vi "Load test file.vi"() -> (1 "Voltaje del detector [V]":dbl[](array[numeric]), 2 "Corriente [mA]":dbl[](array[numeric]), 3 "Voltaje [V]":dbl[](array[numeric]))   [LabVIEW 2020]
uses:
  controls/Graph data --typedef.ctl
  <vilib>/Utility/file.llb/Read Delimited Spreadsheet (DBL).vi
panel:
  out "Eficiencia luminosa-V":cluster{dbl[], dbl[]}(graph) caption="L-V"
  out "Eficiencia de corriente-V":cluster{dbl[], dbl[]}(graph) caption="L-V"
  out "J-V":cluster{dbl[], dbl[]}(graph)
  out "L-V":cluster{dbl[], dbl[]}(graph)
  out "Graph data":T1
  out "Eficiencia luminosa [lm/W]":dbl[](array[numeric])
  out "Eficiencia de corriente [Cd/A]":dbl[](array[numeric])
  out "Luminancia [Cd/m2]":dbl[](array[numeric])
  out "Iluminancia [Lux]":dbl[](array[numeric])
  out "Densidad de corriente [mA/cm2]":dbl[](array[numeric])
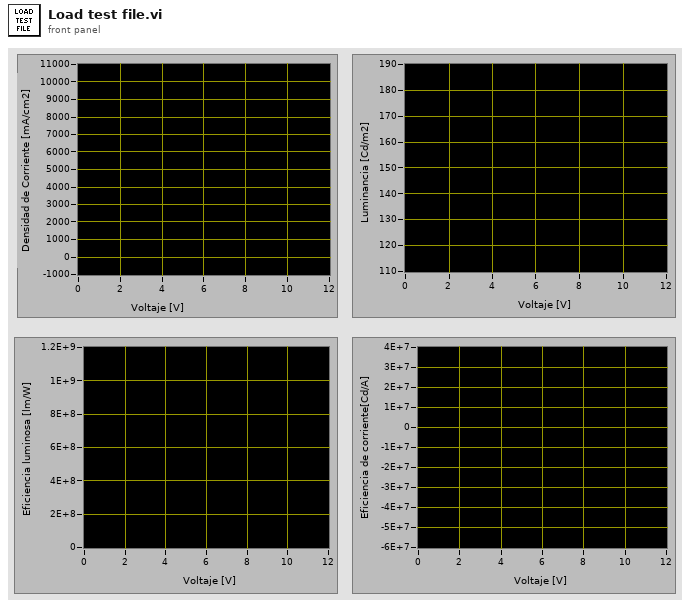
[diagram p1: front panel]
types:
  T1 = typedef "Graph data --typedef.ctl" = cluster{"Voltaje [V]":dbl[], "Corriente [mA]":dbl[], "Densidad de corriente [CD/A]":dbl[], "Iluminancia [Lm/m2]":dbl[], "Luminance [Cd/m2]":dbl[], "Ef corriente [Cd/A]":dbl[], "Ef Luminosa [Cd/W]":dbl[], "V detector [V]":dbl[], "Pin [W]":dbl[]}
  T2 = cluster{"Voltaje [V]":dbl[], "Densidad de corriente [CD/A]":dbl[]}
  T3 = cluster{"Voltaje [V]":dbl[], "Luminance [Cd/m2]":dbl[]}
  T4 = cluster{"Voltaje [V]":dbl[], "Ef corriente [Cd/A]":dbl[]}
  T5 = cluster{"Voltaje [V]":dbl[], "Ef Luminosa [Cd/W]":dbl[]}
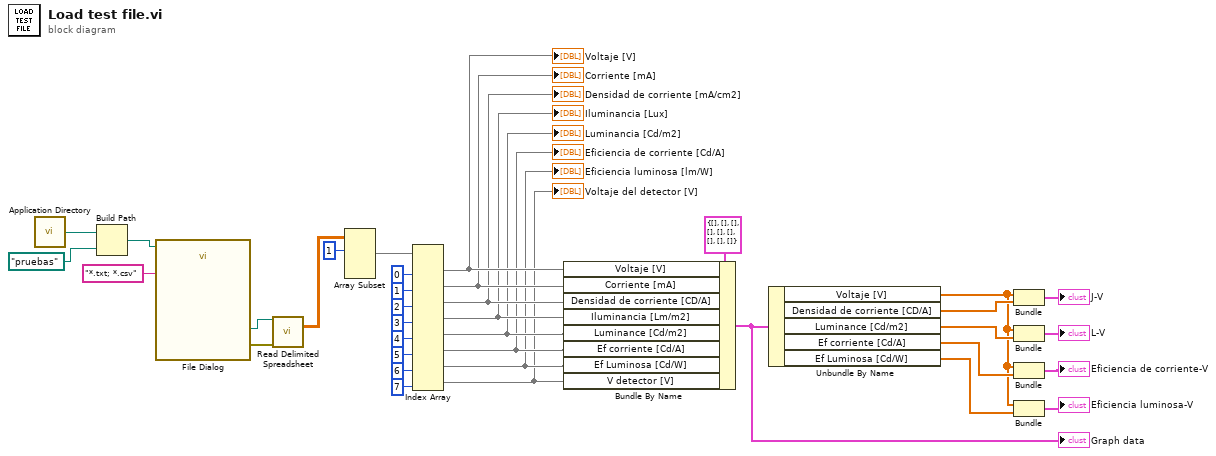
[diagram p0: block diagram]
diagram:
  n1 = call <vilib>:"Application Directory.vi"() -> ("Application Directory"=w36:path)
  n2 = Build Path(base path=w36, name or relative path=path "pruebas") -> (appended path=w34:path)
  n3 = call "File Dialog"("start path"=w34, "pattern (all files)"="*.txt; *.csv") -> ("selected path"=w32:path, "error out"=w29:errorcluster)  [unwired: 10 in, 2 out]
  n4 = call-poly <vilib>:"Read Delimited Spreadsheet.vi"("file path (dialog if empty)"=w32, "error in (no error)"=w29) -> ("all rows"=w31:dbl[][])  [unwired: 8 in, 5 out]
  n5 = Array Subset(array=w31, index (row)=1 ("index")) -> (w28:dbl[][])  [unwired: 3 in]
  n6 = Index Array(array=w28, index (col) #1=0 ("disabled index (col)"), index (col) #2=1 ("index (col)"), index (col) #3=2 ("index (col)"), index (col) #4=3 ("index (col)"), index (col) #5=4 ("index (col)"), index (col) #6=5 ("index (col)"), index (col) #7=6 ("index (col)"), index (col) #8=7 ("index (col)")) -> (element #1=w18:dbl[], element #2=w17:dbl[], element #3=w16:dbl[], element #4=w15:dbl[], element #5=w14:dbl[], element #6=w13:dbl[], element #7=w12:dbl[], element #8=w11:dbl[])  [unwired: 8 in]
  "Voltaje [V]" <- w18
  "Corriente [mA]" <- w17
  "Densidad de corriente [mA/cm2]" <- w16
  "Iluminancia [Lux]" <- w15
  "Luminancia [Cd/m2]" <- w14
  "Eficiencia de corriente [Cd/A]" <- w13
  "Eficiencia luminosa [lm/W]" <- w12
  "Voltaje del detector [V]" <- w11
  n7 = Bundle By Name(cluster=T1 {"Voltaje [V]"=[], "Corriente [mA]"=[], "Densidad de corriente [CD/A]"=[], "Iluminancia [Lm/m2]"=[], "Luminance [Cd/m2]"=[], "Ef corriente [Cd/A]"=[], "Ef Luminosa [Cd/W]"=[], "V detector [V]"=[], "Pin [W]"=[]} ("Graph data"), "Voltaje [V]"=w18, "Corriente [mA]"=w17, "Densidad de corriente [CD/A]"=w16, "Iluminancia [Lm/m2]"=w15, "Luminance [Cd/m2]"=w14, "Ef corriente [Cd/A]"=w13, "Ef Luminosa [Cd/W]"=w12, "V detector [V]"=w11) -> (w10:T1)
  "Graph data" <- w10
  n8 = Unbundle By Name(w10) -> ("Voltaje [V]"=w3:dbl[], "Densidad de corriente [CD/A]"=w9:dbl[], "Luminance [Cd/m2]"=w7:dbl[], "Ef corriente [Cd/A]"=w4:dbl[], "Ef Luminosa [Cd/W]"=w2:dbl[])
  n9 = Bundle("Voltaje [V]"=w3, "Densidad de corriente [CD/A]"=w9) -> (→"J-V":T2)  [unwired: 1 in]
  n10 = Bundle("Voltaje [V]"=w3, "Luminance [Cd/m2]"=w7) -> (→"L-V":T3)  [unwired: 1 in]
  n11 = Bundle("Voltaje [V]"=w3, "Ef corriente [Cd/A]"=w4) -> (→"Eficiencia de corriente-V":T4)  [unwired: 1 in]
  n12 = Bundle("Voltaje [V]"=w3, "Ef Luminosa [Cd/W]"=w2) -> (→"Eficiencia luminosa-V":T5)  [unwired: 1 in]
